vi "Test Process Log Handler Configured.vi"(8 "error in (no error)":errorcluster, 11 "Process Test In":refnum<class "Process Test.lvclass">) -> (0 "error out":errorcluster, 3 "Process Test Out":refnum<class "Process Test.lvclass">)   [LabVIEW 2020, in "Process Test.lvclass"]
uses:
  Process Test.lvclass
  C:/Program Files (x86)/National Instruments/LabVIEW 2020/vi.lib/Astemes/LUnit/Test Case.lvclass
  Mock Log Handler/Mock Log Handler.lvclass
  C:/Git/astemes-triarc-framework/source/Framework/Logging/Logging.lvclass
  Framework/Process/Process.lvclass/Process.ctl
  <vilib>/Astemes/LUnit/Test Case.lvclass/Test Case.ctl
  Framework/Process/Public/Lifecycle/Get Lifecycle State.vi
  Framework/Process/Protected/Messaging/Send Message.vi
  Framework/Process/Private/SubVIs/Wait for finish.vi
  Framework/Process/Private/SubVIs/Set Lifecycle State.vi
  <vilib>/Astemes/LUnit/Set Assertion Type.vi
  <vilib>/Astemes/LUnit/Palette/Pass.vi
  <vilib>/Astemes/LUnit/Palette/Fail.vi
  <vilib>/Utility/error.llb/Clear Errors.vi
  Framework/Process/Private/SubVIs/Handle Debug Data.vi
  <vilib>/Astemes/LUnit/Add test result.vi
  Framework/Logging/Log Debug.vi
  <vilib>/AdvancedString/1D String Array to Delimited String.vi
  <vilib>/Utility/High Resolution Relative Seconds.vi
  <vilib>/Astemes/LUnit/LUnit Record Assertion Result.vi
  <vilib>/Astemes/LUnit/LUnit Aggregate Assertion Results.vi
  <vilib>/Astemes/LUnit/Method Result/LUnit Merge Status.vi
  <vilib>/Astemes/LUnit/LUnit Concatenate result strings.vi
  <vilib>/Utility/error.llb/Error Cluster From Error Code.vi
  Framework/Process/Public/Read Name.vi
  Framework/Process/Process.lvclass
  Process Test.lvclass/Process Test.ctl
  <vilib>/Astemes/LUnit/Test Case.lvclass
  C:/Git/astemes-triarc-framework/source/Framework/Base/Base.lvclass
  C:/Git/astemes-triarc-framework/source/Framework Test Suite/Mock Log Handler/Mock Log Handler.lvclass
  C:/Git/astemes-triarc-framework/source/Framework Test Suite/Base Class Test/Base Test.lvclass
  C:/Git/astemes-triarc-framework/source/Framework Test Suite/Process Test/Process Test.lvclass
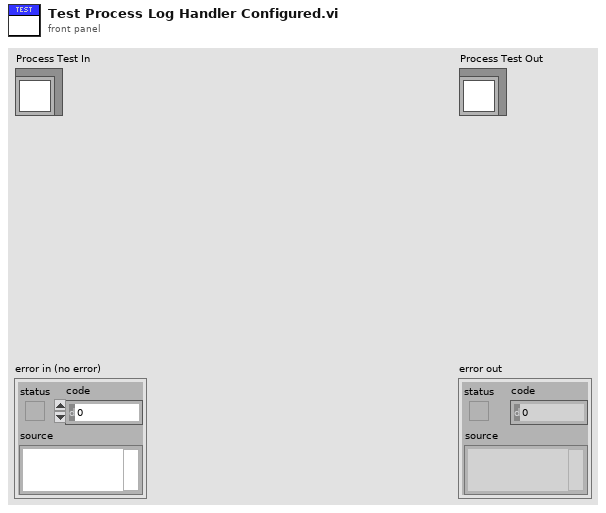
[diagram p1: front panel]
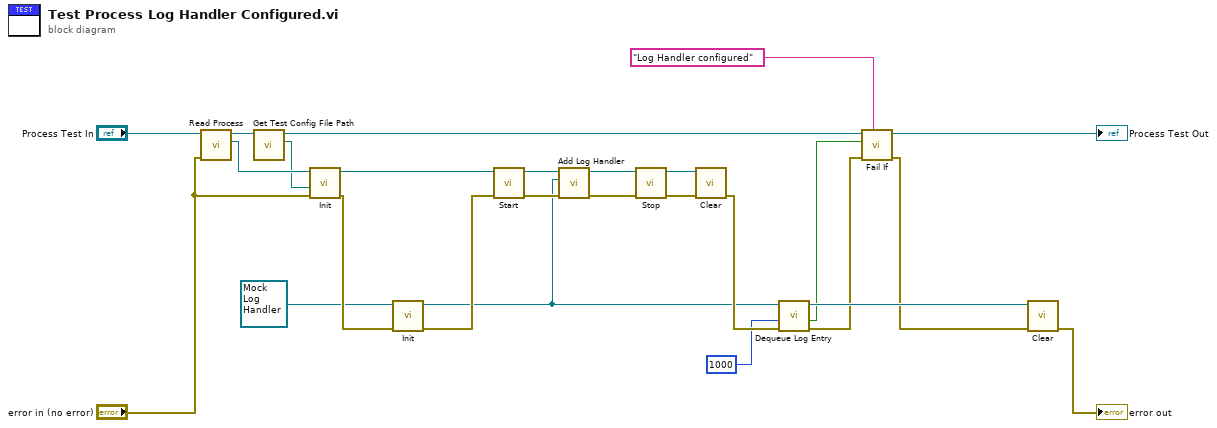
[diagram p0: block diagram]
diagram:
  n1 = call "Read Process.vi"("error in (no error)"="error in (no error)", "Process Test in"="Process Test In") -> ("Process.lvclass"=w14:refnum<class "Process.lvclass">, "Process Test out"=w13:refnum<class "Process Test.lvclass">)  [unwired: 7 in, 1 out]
  n2 = call "Get Test Config File Path.vi"("Process Test In"=w13) -> ("Test config path"=w1:path, "Process Test Out"=w2:refnum<class "Process Test.lvclass">)  [unwired: 8 in, 1 out]
  n3 = call-dynamic "Init.vi"("error in (no error)"="error in (no error)", "Config File Path"=w1, "Process In"=w14) -> ("error out"=w25:errorcluster, "Process Out"=w5:refnum<class "Process.lvclass">)  [unwired: 7 in]
  n4 = call-dynamic "Init.vi"("error in (no error)"=w25, "Mock Log Handler In"=refnum<class "Mock Log Handler.lvclass"> refnum ("Mock Log Handler.lvclass")) -> ("error out"=w21:errorcluster, "Mock Log Handler Out"=w3:refnum<class "Mock Log Handler.lvclass">)  [unwired: 8 in]
  n5 = call "Start.vi"("error in (no error)"=w21, "Process In"=w5) -> ("error out"=w6:errorcluster, "Process Out"=w4:refnum<class "Process.lvclass">)  [unwired: 7 in, 1 out]
  n6 = call "Add Log Handler.vi"("error in (no error)"=w6, "Log Handler"=w3, "Process In"=w4) -> ("error out"=w22:errorcluster, "Process Out"=w23:refnum<class "Process.lvclass">)  [unwired: 7 in]
  n7 = call "Stop.vi"("error in (no error)"=w22, "Process In"=w23) -> ("error out"=w8:errorcluster, "Process Out"=w7:refnum<class "Process.lvclass">)  [unwired: 7 in, 1 out]
  n8 = call-dynamic "Clear.vi"("error in (no error)"=w8, "Process In"=w7) -> ("error out"=w18:errorcluster)  [unwired: 9 in]
  n9 = call "Dequeue Log Entry.vi"("error in (no error)"=w18, "timeout in ms (-1)"=1000, "Mock Log Handler in"=w3) -> ("error out"=w17:errorcluster, "timed out?"=w9:bool, "Mock Log Handler out"=w20:refnum<class "Mock Log Handler.lvclass">)  [unwired: 5 in, 1 out]
  n10 = call <vilib>:"Fail If.vi"("Description"="Log Handler configured", "error in (no error)"=w17, "Fail?"=w9, "LUnit Test Case In"=w2) -> ("error out"=w16:errorcluster, "LUnit Test Case Out"=→"Process Test Out":refnum<class "Process Test.lvclass">)  [unwired: 6 in]
  n11 = call-dynamic "Clear.vi"("error in (no error)"=w16, "Mock Log Handler In"=w20) -> ("error out"=→"error out":errorcluster)  [unwired: 9 in]
